vi "ToRepo.vi"(8 "error in":errorcluster, 9 "to repo cluster":T1, 10 "repository in":refnum<class "NISE_CEF_Repository.lvclass">, 11 "node in":refnum<class "Systems.lvclass">) -> (0 "error out":errorcluster, 2 "repository out":refnum<class "NISE_CEF_Repository.lvclass">, 3 "node out":refnum<class "Systems.lvclass">)   [LabVIEW 2013, in "PL Framework Configuration Tool.lvlib" / "Systems.lvclass"]
doc: "Transfers the information from the tree node into the repo. How it is stored in the repo depends on the Repo. For children of NISE_CEF_serializable node.lvclass, the parent method must be called to maintain the chain of serialization. If it is not called, the repo generation will fail."
uses:
  Systems.lvclass
  <vilib>/NI/Configuration Framework/Repository/NISE_CEF_Repository.lvclass
  <vilib>/NI/Configuration Framework/Node/ToRepoCluster.ctl
  Systems.lvclass/Systems.ctl
  Framework Configuration Classes/system configuration/PL_System Configuration.lvclass/PL_System Configuration.ctl
  TBM Configuration Node/TBM Configuration Node.lvclass
  Framework Configuration Classes/system configuration/PL_System Configuration.lvclass
  <vilib>/NI/Configuration Framework/Node/NISE_CEF_Node.lvclass
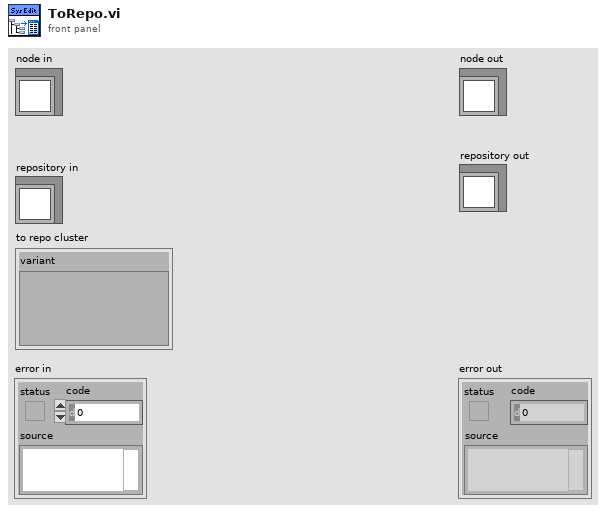
[diagram p1: front panel]
types:
  T1 = typedef "NISE_CEF_Node.lvclass/ToRepoCluster.ctl" = cluster{"variant":variant}
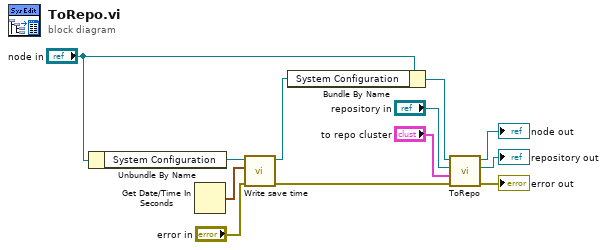
[diagram p0: block diagram]
diagram:
  n1 = Unbundle By Name("node in") -> ("System Configuration"=w5:refnum<class "PL_System Configuration.lvclass">)
  n2 = Get Date/Time In Seconds() -> (seconds since 1Jan1904=w1:timestamp)
  n3 = call "Write save time.vi"("error in"="error in", "save time"=w1, "PL_System Configuration in"=w5) -> ("error out"=w3:errorcluster, "PL_System Configuration out"=w4:refnum<class "PL_System Configuration.lvclass">)  [unwired: 7 in]
  n4 = Bundle By Name(cluster="node in", "System Configuration"=w4) -> (w6:refnum<class "Systems.lvclass">)
  n5 = call-parent "ToRepo.vi"("error in"=w3, "to repo cluster"="to repo cluster", "repository in"="repository in", "node in"=w6) -> ("error out"=→"error out":errorcluster, "repository out"=→"repository out":refnum<class "NISE_CEF_Repository.lvclass">, "node out"=→"node out":refnum<class "Systems.lvclass">)  [unwired: 5 in]
